vi "ChangeStrCnstValue.vi"(0 "VI Path":path, 5 "Label Name":string, 7 "New Value":string, 11 "Error In":errorcluster) -> (15 "Error Out":errorcluster)   [LabVIEW 2019, in "Drona.lvlib"]
doc: "This VI changes the string constant value to new value of another VI based on the label"
uses:
  Drona.lvlib
  <vilib>/Utility/traverseref.llb/TRef TravTarget.ctl
  <vilib>/Utility/traverseref.llb/VI Scripting - Traverse.lvlib
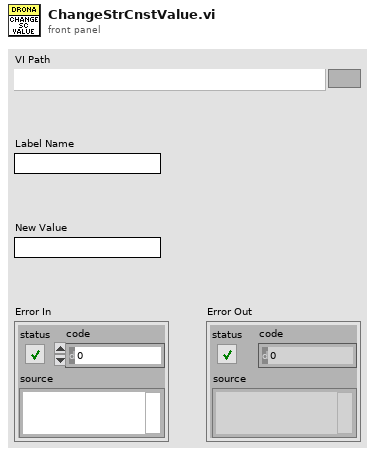
[diagram p1: front panel]
types:
  T1 = typedef "TRef TravTarget.ctl" = enum16{"FP", "BD", "Other"}
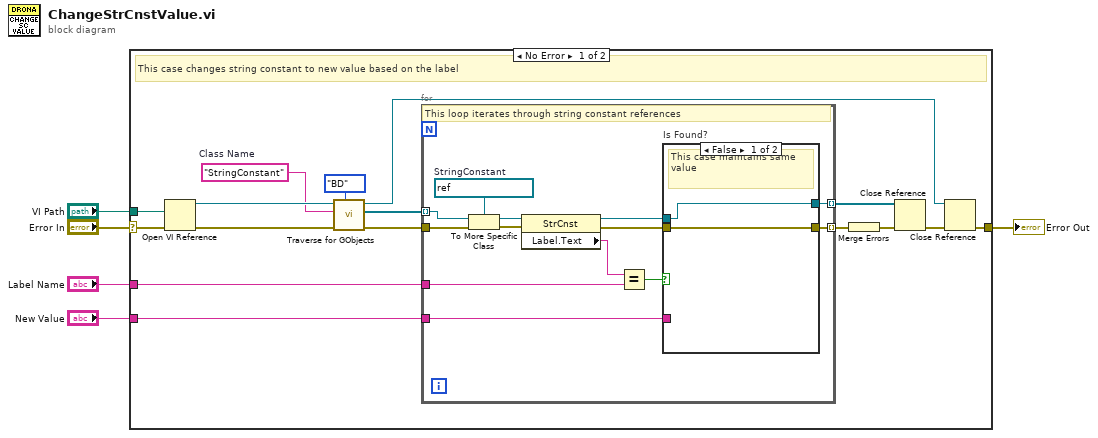
[diagram p0: block diagram]
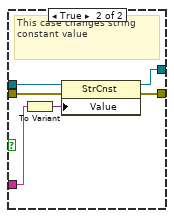
[diagram p2: hidden frame]
diagram:
  n1 = case shown="No Error" "Error In" {
    selector: "Error In" -> [w21 w43]
    tunnel: "VI Path" -> [w20 _]
    tunnel: "Label Name" -> [w14 _]
    tunnel: "New Value" -> [w13 _]
    tunnel: [w7 w43] -> w1
    frame No Error {
      w17 = "StringConstant"  # Class Name
      # "This case changes string constant to new value based on the label"
      n2 = Open VI Reference(vi path=w20, error in (no error)=w21) -> (vi reference=w19:refnum<vi>, error out=w18:errorcluster)  [unwired: 4 in]
      n3 = call <vilib>:"Traverse for GObjects.vi"("Traverse Target"=TRef_TravTarget."BD", "error in (no error)"=w18, "Class Name"=w17, "VI Refnum"=w19) -> ("error out"=w16:errorcluster, "References"=w15:refnum<vi>[], "dup VI Refnum"=w8:refnum<vi>)  [unwired: 4 in, 1 out]
      n4 = for {
        tunnel: w16 -> [w32]
        tunnel: w15 -> [w34] mode=indexing
        tunnel: w14 -> [w28]
        tunnel: [w25] -> w12 mode=indexing
        tunnel: w13 -> [w23]
        tunnel: [w22] -> w10 mode=indexing
        w30 = refnum<vi> refnum  # StringConstant
        # "This loop iterates through string constant references"
        n5 = To More Specific Class(target class=w30, reference=w34, error in=w32) -> (specific class reference=w33:refnum<vi>, error out=w31:errorcluster)
        n6 = property class="StrCnst"(reference=w33, error in=w31) -> (reference out=w24:refnum<vi>, error out=w27:errorcluster, "Label.Text"=w29:string)
        n7 = Equal?(x=w29, y=w28) -> (x = y?=w26:bool)
        n8 = case "Is Found?" shown="False" w26 {
          tunnel: w27 -> [w35 w42]
          tunnel: [w35 w41] -> w25
          tunnel: w24 -> [w36 w40]
          tunnel: w23 -> [_ w39]
          tunnel: [w36 w38] -> w22
          frame False {
            # "This case maintains same value"
          }
          frame True {
            # "This case changes string constant value"
            n9 = To Variant(anything=w39) -> (Variant=w37:variant)
            n10 = property class="StrCnst"(reference=w40, error in=w42, "Value"=w37) -> (reference out=w38:refnum<vi>, error out=w41:errorcluster)
          }
        }
      }
      n11 = Merge Errors(w12) -> (w11:errorcluster)
      n12 = Close Reference(reference=w10, error in (no error)=w11) -> (error out=w9:errorcluster)
      n13 = Close Reference(reference=w8, error in (no error)=w9) -> (error out=w7:errorcluster)
    }
    frame Error {
    }
  }
  "Error Out" <- w1
